vi "xnet_canopen_read_batch.vi"(8 "error in (no error)":errorcluster, 10 "OD Batch in":refnum<class "OD Batch.lvclass">, 11 "xnet_co_handle_in":u64) -> (0 "error out":errorcluster, 2 "OD Batch":refnum<class "OD Batch.lvclass">, 3 "xnet_co_handle":u64)   [LabVIEW 2023, in "xnet_canopen.lvlib"]
uses:
  xnet_canopen.lvlib
  OD Batch/OD Batch.lvclass
  OD Batch/OD Batch.lvclass/OD Batch.ctl
  <vilib>/Utility/error.llb/Error Cluster From Error Code.vi
  OD Batch/Read Batch OD By Array Index.vi
  OD Batch/Read Batch OD By Array Index - bool.vi
  OD Batch/Read Batch OD By Array Index - i8.vi
  OD Batch/Read Batch OD By Array Index - i16.vi
  OD Batch/Read Batch OD By Array Index - i32.vi
  OD Batch/Read Batch OD By Array Index - u8.vi
  OD Batch/Read Batch OD By Array Index - u16.vi
  OD Batch/Read Batch OD By Array Index - u32.vi
  OD Batch/Read Batch OD By Array Index - f32.vi
  OD Batch/Read Batch OD By Array Index - string.vi
  OD Batch/Read Batch OD By Array Index - bytes.vi
  OD Batch/Read Batch OD By Array Index - f64.vi
  OD Batch/Read Batch OD By Array Index - i64.vi
  OD Batch/Read Batch OD By Array Index - u64.vi
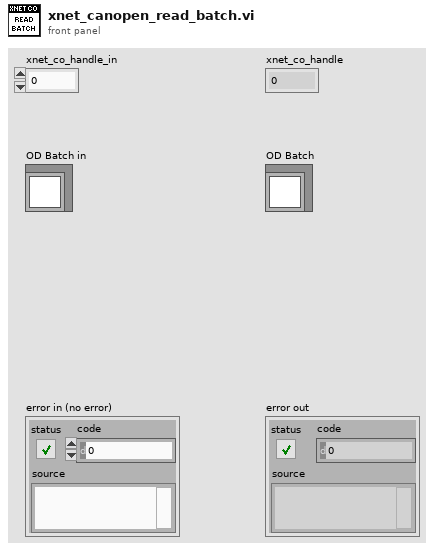
[diagram p1: front panel]
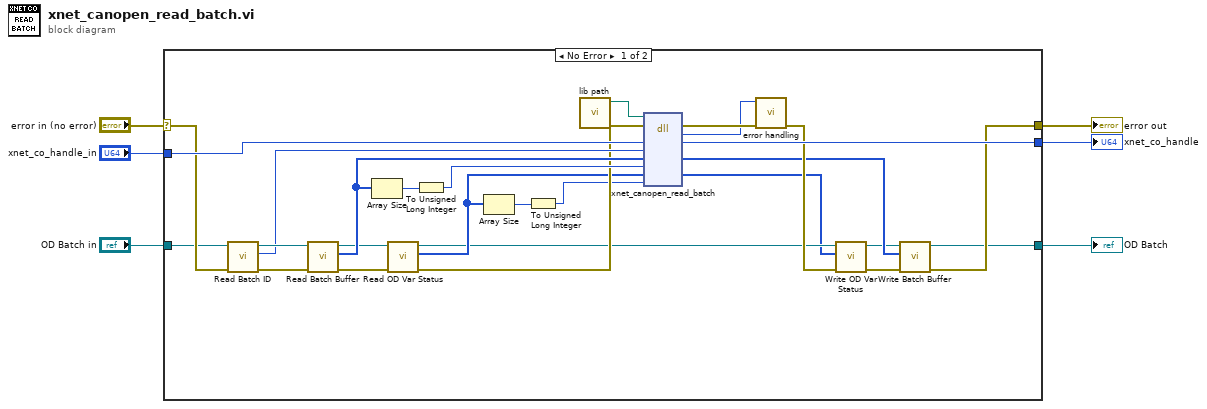
[diagram p0: block diagram]
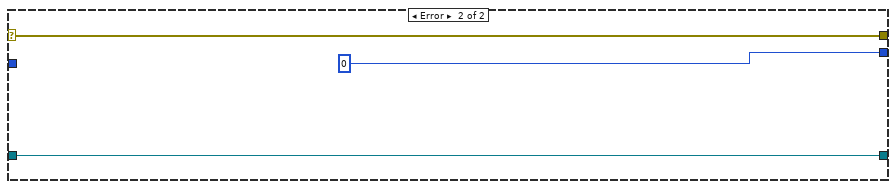
[diagram p2: hidden frame]
diagram:
  n1 = case shown="No Error" "error in (no error)" {
    selector: "error in (no error)" -> [w28 w36]
    tunnel: [w8 w36] -> w5
    tunnel: [w30 u64 0 ("phandle")] -> w4
    tunnel: "xnet_co_handle_in" -> [w29 _]
    tunnel: "OD Batch in" -> [w26 w34]
    tunnel: [w7 w34] -> w1
    frame No Error {
      n2 = call "Read Batch ID.vi"("error in (no error)"=w28, "OD Batch in"=w26) -> ("error out"=w27:errorcluster, "Batch ID"=w24:u32, "OD Batch out"=w25:refnum<class "OD Batch.lvclass">)  [unwired: 7 in]
      n3 = call "Read Batch Buffer.vi"("error in (no error)"=w27, "OD Batch in"=w25) -> ("error out"=w23:errorcluster, "Batch Buffer"=w22:u8[], "OD Batch out"=w18:refnum<class "OD Batch.lvclass">)  [unwired: 7 in]
      n4 = Array Size(array=w22) -> (size(s)=w21:i32)
      n5 = call "Read OD Var Status.vi"("error in (no error)"=w23, "OD Batch in"=w18) -> ("error out"=w19:errorcluster, "OD Var Status"=w17:i32[], "OD Batch out"=w13:refnum<class "OD Batch.lvclass">)  [unwired: 7 in]
      n6 = To Unsigned Long Integer(number=w21) -> (unsigned 32bit integer=w20:u32)
      n7 = Array Size(array=w17) -> (size(s)=w16:i32)
      n8 = To Unsigned Long Integer(number=w16) -> (unsigned 32bit integer=w15:u32)
      n9 = call "lib path.vi"() -> ("lib path"=w33:path)  [unwired: 11 in]
      n10 = dll-call lib="?" fn="xnet_canopen_read_batch"(path in=w33, error in=w19, "handle"=w29, "batch_id"=w24, "buffer"=w22, "bufsize"=w20, "entry_status"=w17, "entry_cnt"=w15) -> (error out=w32:errorcluster, "return type"=w31:i32, "handle"=w30:u64, "buffer"=w11:u8[], "entry_status"=w12:i32[])  [unwired: 4 in, 1 out]
      n11 = call "error handling.vi"("error in (no error)"=w32, "return val"=w31) -> ("error out"=w14:errorcluster)  [unwired: 9 in]
      n12 = call "Write OD Var Status.vi"("error in (no error)"=w14, "OD Var Status"=w12, "OD Batch in"=w13) -> ("error out"=w9:errorcluster, "OD Batch out"=w10:refnum<class "OD Batch.lvclass">)  [unwired: 7 in]
      n13 = call "Write Batch Buffer.vi"("error in (no error)"=w9, "Batch Buffer"=w11, "OD Batch in"=w10) -> ("error out"=w8:errorcluster, "OD Batch out"=w7:refnum<class "OD Batch.lvclass">)  [unwired: 7 in]
    }
    frame Error {
    }
  }
  "error out" <- w5
  "xnet_co_handle" <- w4
  "OD Batch" <- w1
